vi "RemoteVI Start Landing Page.vi"(1 "whole network?":bool, 2 "token":string, 5 "port":u16=8088, 11 "error in":errorcluster) -> (4 "URL":string, 6 "port out":u16, 15 "error out":errorcluster)   [LabVIEW 2020, in "RemoteVI.lvlib"]
doc: "Starts RemoteVI Server's landing page: RemoteVI Landing Server.vi (found next to this VI) launched like a share (RemoteVI Launch Share.vi with loop VI), so it also needs its own random token and listens on 127.0.0.1 unless whole network? is TRUE. When port is in use (error 60) the next port is tried, up to 20 ports; port out is the one that listens. Stop it with RemoteVI Stop.vi and port out."
uses:
  RemoteVI.lvlib
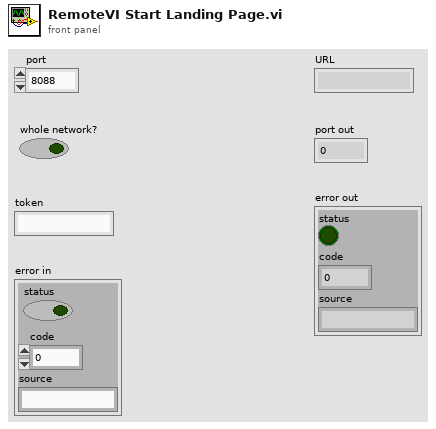
[diagram p1: front panel]
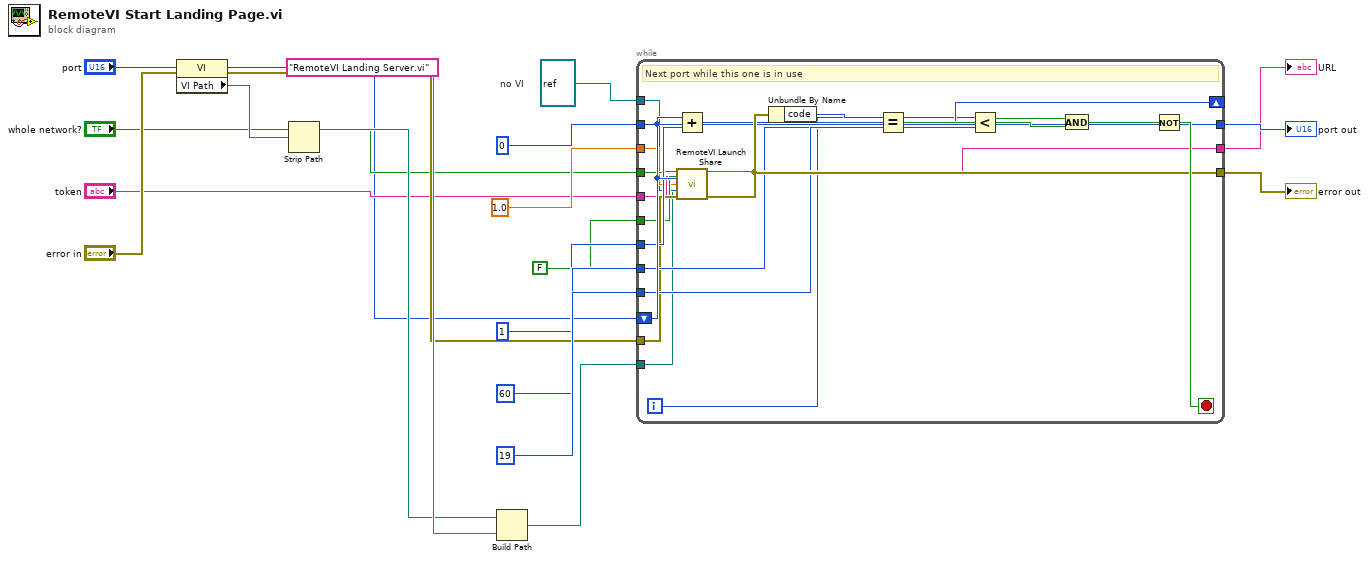
[diagram p0: block diagram]
diagram:
  w10 = refnum<vi> refnum  # no VI
  n1 = property class="VI"(error in="error in") -> (error out=w5:errorcluster, "VI Path"=w6:path)  [unwired: 1 in, 1 out]
  n2 = Strip Path(path=w6) -> (stripped path=w7:path)  [unwired: 1 out]
  n3 = Build Path(base path=w7, name or relative path="RemoteVI Landing Server.vi") -> (appended path=w9:path)
  n4 = while {
    tunnel: w10 -> [w22]
    tunnel: u64 0 -> [w23]
    tunnel: 1.0 -> [w24]
    tunnel: "whole network?" -> [w25]
    tunnel: "token" -> [w26]
    tunnel: FALSE -> [w27]
    tunnel: u16 1 -> [w29]
    tunnel: 60 -> [w30]
    tunnel: 19 -> [w31]
    shift-right: [w33] -> _
    shift-left: "port" -> [w32]
    tunnel: w5 -> [w28]
    tunnel: [w32] -> w18
    tunnel: w9 -> [w21]
    tunnel: [w34] -> w17
    tunnel: [w35] -> w19
    i -> [w20]
    stop <- w40 stop-if-true
    # "Next port while this one is in use"
    n5 = Add(x=w32, y=w29) -> (x+y=w33:u16)
    n6 = call "RemoteVI Launch Share.vi"("VI"=w22, "whole network?"=w25, "token"=w26, "view only?"=w27, "port"=w32, "fps"=w24, "window"=w23, "loop VI"=w21, "error in"=w28) -> ("URL"=w34:string, "error out"=w35:errorcluster)  [unwired: 5 in]
    n7 = Unbundle By Name(w35) -> ("code"=w36:i32)
    n8 = Equal?(x=w36, y=w30) -> (x = y?=w37:bool)
    n9 = Less?(x=w20, y=w31) -> (x < y?=w38:bool)
    n10 = And(x=w37, y=w38) -> (x .and. y?=w39:bool)
    n11 = Not(x=w39) -> (.not. x?=w40:bool)
  }
  "URL" <- w17
  "port out" <- w18
  "error out" <- w19
